vi "IMU Get Yaw Portrait.vi"(7 "Set Yaw Angle":dbl=nan, 8 "error in (no error)":errorcluster, 10 "Units":enum16{"Radians", "Degrees"}(ring)) -> (0 "error out":errorcluster, 2 "timestamp out":i64, 3 "yaw":dbl(graph))   [LabVIEW 2023, in "MrcLib.lvlib"]
doc: "Return the yaw of the built-in sensor in the indicated units assuming the controller is mounted vertical with narrow edge parallel to the ground (less common). To align with a existing coordinate system, make a call passing in the expected alignment angle."
uses:
  <vilib>/MRC/MrcLib.lvlib
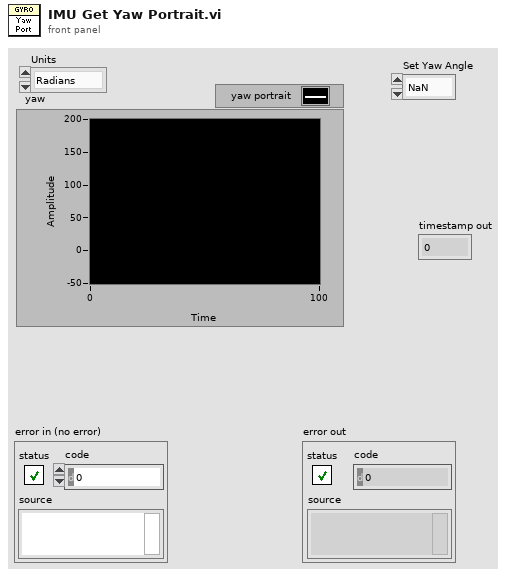
[diagram p1: front panel]
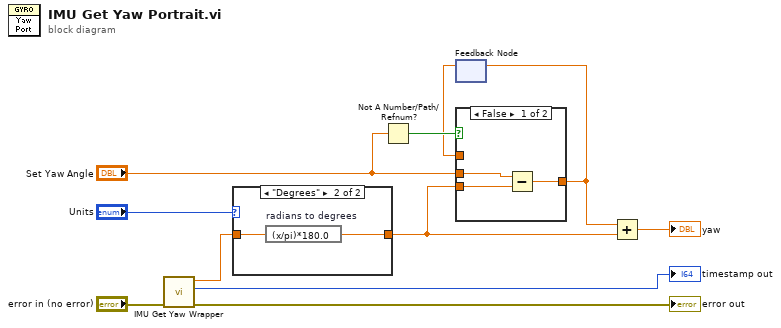
[diagram p0: block diagram]
diagram:
  n1 = call-poly <vilib>:"IMU Get Yaw Wrapper.vi"("error in (no error)"="error in (no error)") -> ("error out"=→"error out":errorcluster, "timestamp out"=→"timestamp out":i64, "yaw out"=w8:dbl)  [unwired: 7 in, 1 out]
  n2 = case shown="\"Degrees\"" "Units" {
    tunnel: w8 -> [w12 w14]
    tunnel: [w12 w13] -> w2
    frame "Radians", Default {
    }
    frame "Degrees" {
      n3 = expression code="(x/pi)*180.0" "radians to degrees"(w14) -> (w13:dbl)
    }
  }
  n4 = Not A Number/Path/Refnum?(number/path/refnum="Set Yaw Angle") -> (NaN/Path/Refnum?=w6:bool)
  n5 = feedback #1() -> (w5:dbl)  [unwired: 1 in]
  n6 = case shown="False" w6 {
    tunnel: w2 -> [w17 _]
    tunnel: "Set Yaw Angle" -> [w16 _]
    tunnel: [w15 w18] -> w4
    tunnel: w5 -> [_ w18]
    frame False {
      n7 = Subtract(x=w16, y=w17) -> (x-y=w15:dbl)
    }
    frame True {
    }
  }
  n8 = feedback-in #1(w4) -> ()
  n9 = Add(x=w4, y=w2) -> (x+y=→"yaw":dbl)
